vi "FlatToRichauth_RefreshTokenResponse.vi"(5 "OutputClusterType":T1, 11 "InputCluster":T2) -> (3 "OutputCluster":T1)   [LabVIEW 2020, in "grpc-auth_client.lvlib"]
uses:
  grpc-auth_client.lvlib
  auth_RefreshTokenResponse_Flat.ctl
  auth_RefreshTokenResponse.ctl
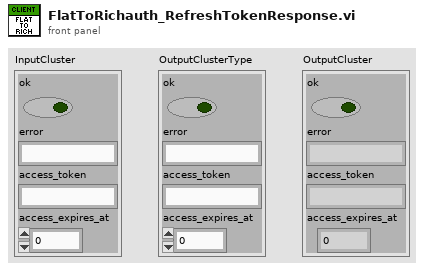
[diagram p1: front panel]
types:
  T1 = typedef "grpc-auth_client.lvlib/auth_RefreshTokenResponse.ctl" = cluster{"ok":bool, "error":string, "access_token":string, "access_expires_at":i64}
  T2 = typedef "grpc-auth_client.lvlib/auth_RefreshTokenResponse_Flat.ctl" = cluster{"ok":bool, "error":string, "access_token":string, "access_expires_at":i64}
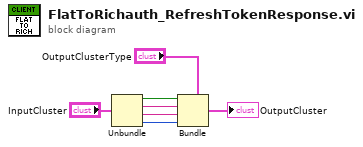
[diagram p0: block diagram]
diagram:
  n1 = Unbundle "Unbundle"("InputCluster") -> ("ok"=w4:bool, "error"=w3:string, "access_token"=w2:string, "access_expires_at"=w1:i64)
  n2 = Bundle "Bundle"(cluster="OutputClusterType", "ok"=w4, "error"=w3, "access_token"=w2, "access_expires_at"=w1) -> (→"OutputCluster":T1)
